vi "query Modulation.vi"(8 "error in (no error)":errorcluster, 11 "LTE in":refnum<class "LTE.lvclass">) -> (0 "error out":errorcluster, 2 "Modulation":T1, 3 "LTE out":refnum<class "LTE.lvclass">)   [LabVIEW 2023, in "ANRITSU Call Box.lvlib" / "LTE.lvclass"]
uses:
  LTE.lvclass
  LTE.lvclass/LTE.ctl
  ANRITSU Call Box.lvlib
  Type Definition/LTE Modulation Type.ctl
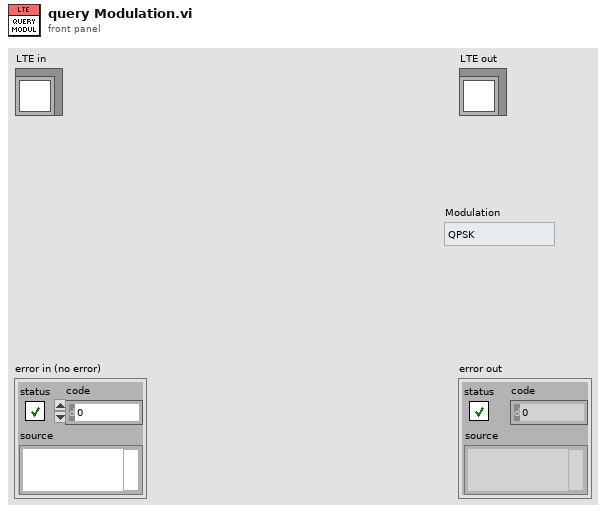
[diagram p1: front panel]
types:
  T1 = typedef "ANRITSU Call Box.lvlib/LTE Modulation Type.ctl" = enum16{"QPSK", "16QAM", "64QAM", "256QAM"}
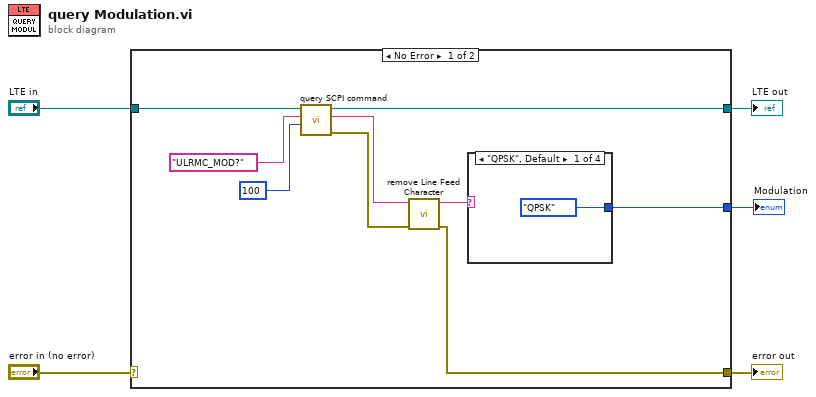
[diagram p0: block diagram]
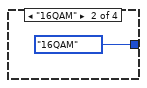
[diagram p2: hidden frame]
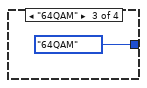
[diagram p3: hidden frame]
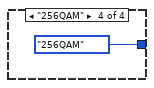
[diagram p4: hidden frame]
diagram:
  n1 = case shown="No Error" "error in (no error)" {
    selector: "error in (no error)" -> [_ w20]
    tunnel: [w6 w20] -> w4
    tunnel: [w8 w19] -> w2
    tunnel: "LTE in" -> [w14 w19]
    tunnel: [w7 _] -> w1
    frame No Error {
      n2 = call "query SCPI command.vi"("Read Buffer Length"=u32 100, "SCPI Command"="ULRMC_MOD?", "LTE in"=w14) -> ("error out"=w10:errorcluster, "Read Buffer String"=w11:string, "LTE out"=w8:refnum<class "LTE.lvclass">)  [unwired: 6 in]
      n3 = call "remove Line Feed Character.vi"("error in"=w10, "Query String"=w11) -> ("error out"=w6:errorcluster, "Line Feed Removed String"=w9:string)  [unwired: 8 in]
      n4 = case shown="\"QPSK\", Default" w9 {
        tunnel: [LTE_Modulation_Type."QPSK" ("Modulation 2") LTE_Modulation_Type."16QAM" ("Modulation 2") LTE_Modulation_Type."64QAM" ("Modulation 2") LTE_Modulation_Type."256QAM" ("Modulation 2")] -> w7
        frame "QPSK", Default {
        }
        frame "16QAM" {
        }
        frame "64QAM" {
        }
        frame "256QAM" {
        }
      }
    }
    frame Error {
    }
  }
  "error out" <- w4
  "LTE out" <- w2
  "Modulation" <- w1
